vi "Variables glob EUROTHERM.vi"() -> ()   [LabVIEW 2022 SP3]
panel:
  in  "Modif en cours":bool
  in  "Donnees Alarmes sur mesure":cluster{"AL sur mes 1COM":string[][]}[](array[cluster])
  in  "Refnum appel suivi AL":refnum<vi>
  out "Date alarme":timestamp
  out "message alarme":string
  in  "AL OK":cluster{"AL OK 1 COM":u16[]}[](array[cluster]) {"AL OK 1 COM" items=["data = AL", "data pas nombre", "data diff. AL"]}
  out "probleme observe":string
  out "Nb reg run":u8[](array[numeric])
  out "Nb reg acqui":u8[](array[numeric])
  in  "Ports COM REG run":refnum<visa-resource-name>[](array[refnum])
  in  "Ports COM REG acqui":refnum<visa-resource-name>[](array[refnum])
  out "Alarmes envoyees reg acqui":cluster{"alarmes 1COM reg":string[][]}[](array[cluster])
  out "Adresses regs run":cluster{"Adresses run 1COM reg":u16[]}[](array[cluster])
  out "Noms voies regs select run":cluster{"Noms voies select run 1COM":string[]}[](array[cluster])
  out "Select regs run":cluster{"Sélect run 1COM reg":bool[]}[](array[cluster])
  in  "Dernieres donnees regs":cluster{"Dernieres donnees 1COM":string[][]}[](array[cluster])
  out "Select regs acqui":cluster{"Select acqui 1COM reg":bool[]}[](array[cluster])
  out "Noms voies regs select acqui":T1(array[cluster])=[{"Noms voies select acqui 1COM"=["reg 1-1", "reg 1-2"]}, {"Noms voies select acqui 1COM"=["reg 2-1", "reg 2-2"]}]
  out "Adresses regs acqui":cluster{"Adresses acqui 1COM reg":u16[]}[](array[cluster])
  out "Noms voies regs dispo":cluster{"Noms voies dispo 1COM":string[]}[](array[cluster])
  out "Adresses regs dispo":cluster{"Adresses 1COM reg":u16[]}[](array[cluster])
  out "Nb reg dispo":u8[](array[numeric])
  in  "REG":bool
  out "semaphores EUROTH":T2[](array[typedef])
  in  "Ports COM REG dispo":refnum<visa-resource-name>[](array[refnum])
  # "parmi regs dispo"
  # "parmi reg acqui"
  # "OP"
  # "Mesure"
  # "Consigne"
  # "Sécurité"
  # "Alarme basse"
  # "Alarme haute"
  # "Alarme basse"
  # "Alarme haute"
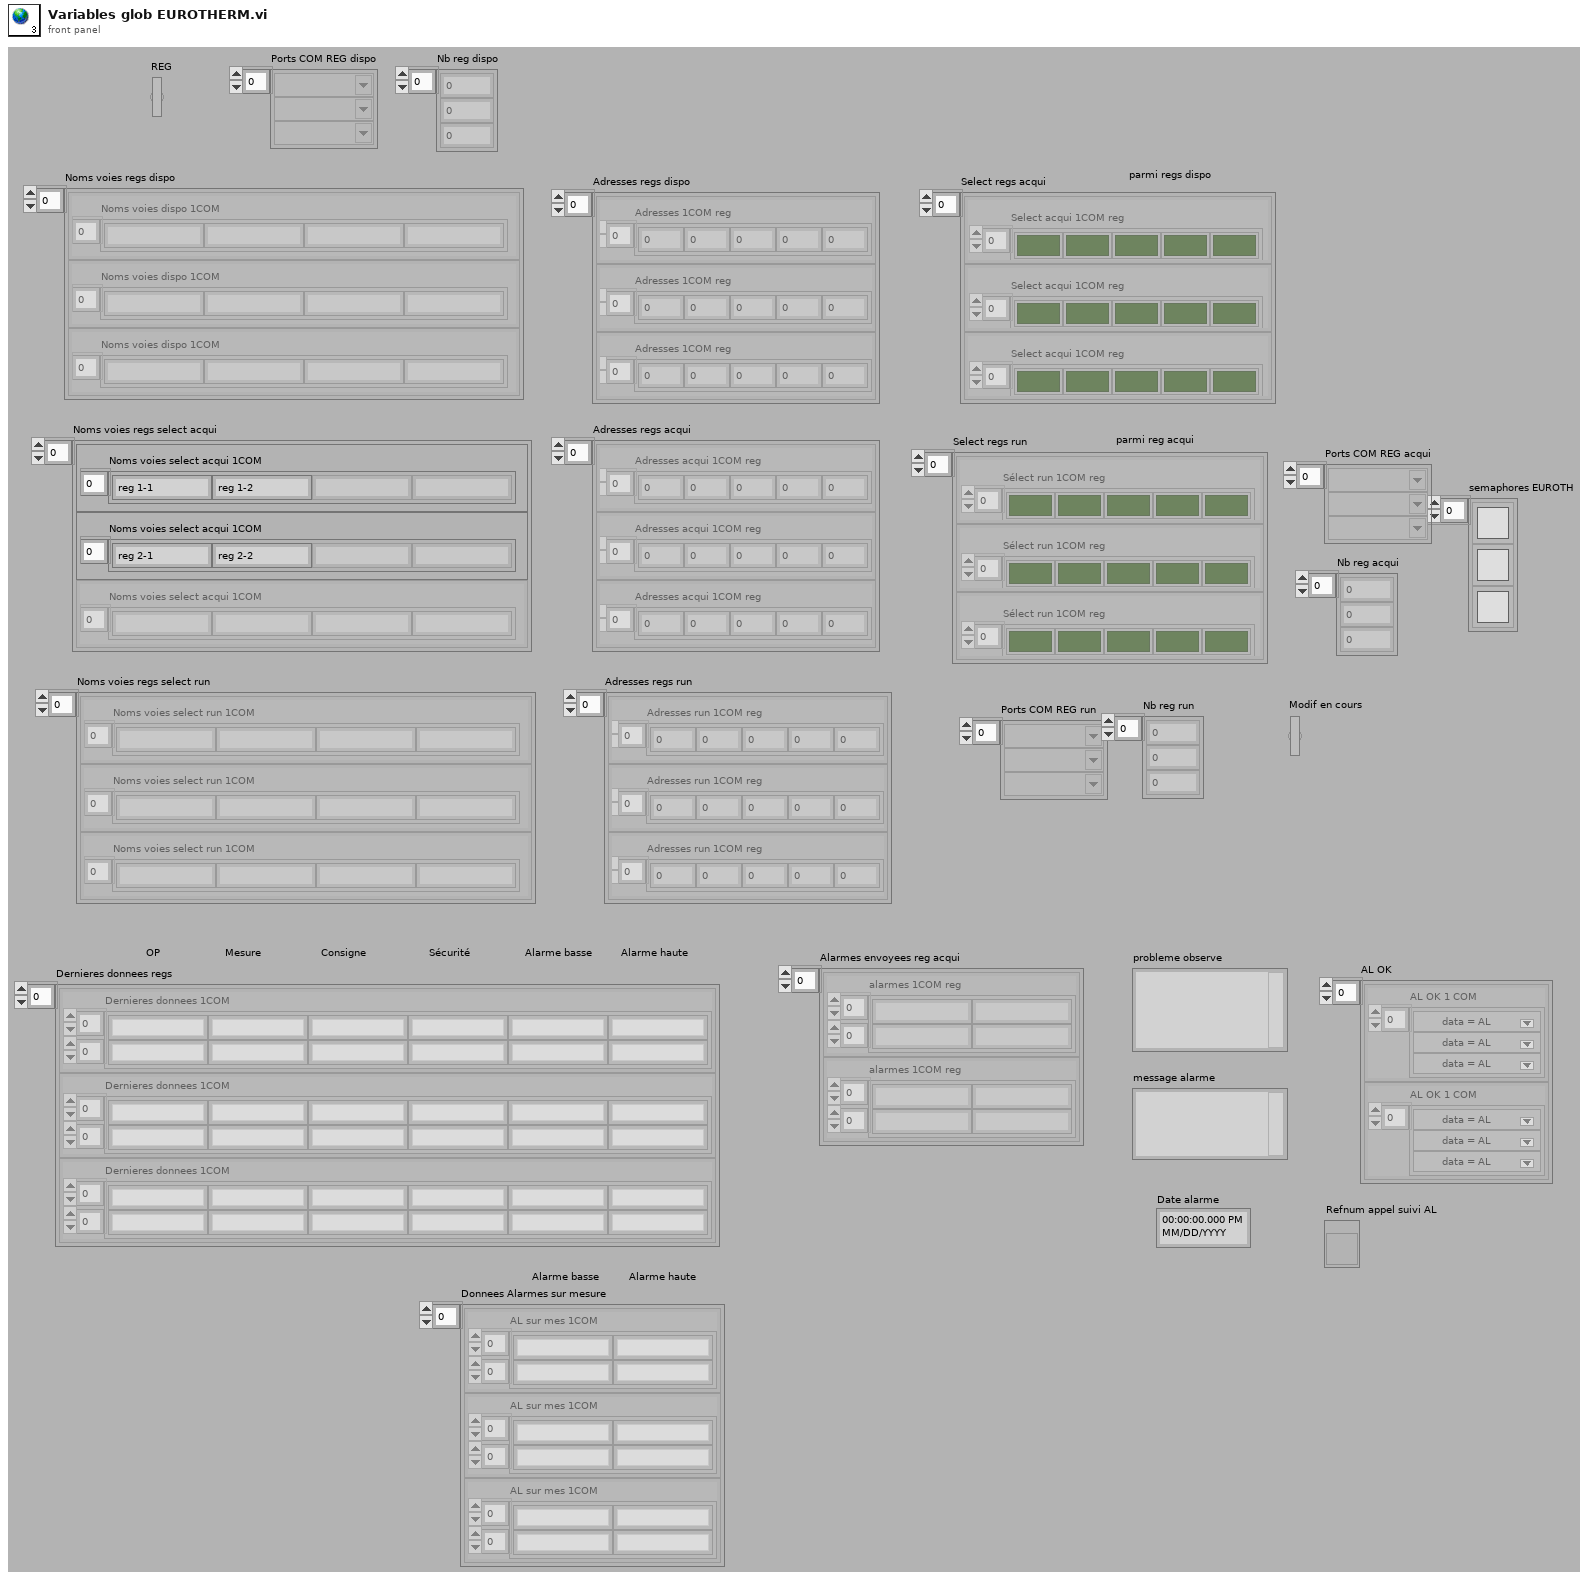
[diagram p1: front panel]
types:
  T1 = cluster{"Noms voies select acqui 1COM":string[]}[]
  T2 = typedef "Semaphore RefNum" = refnum<k1>
diagram:
